vi "Run Tests in Active Project.vi"(10 "Virtual Folder (empty: \"My Computer\")":string) -> ()   [LabVIEW 2020]
uses:
  subVIs/Run Tests (Project).vi
  Caraya.lvlib
panel:
  out "error out":errorcluster
  # "CARAYA Run Active Project's Unit Tests\n\nThis tool will run all Caraya Unit Tests found in the active project."
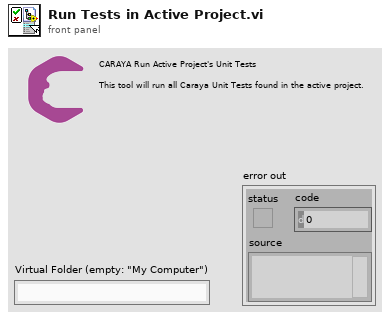
[diagram p1: front panel]
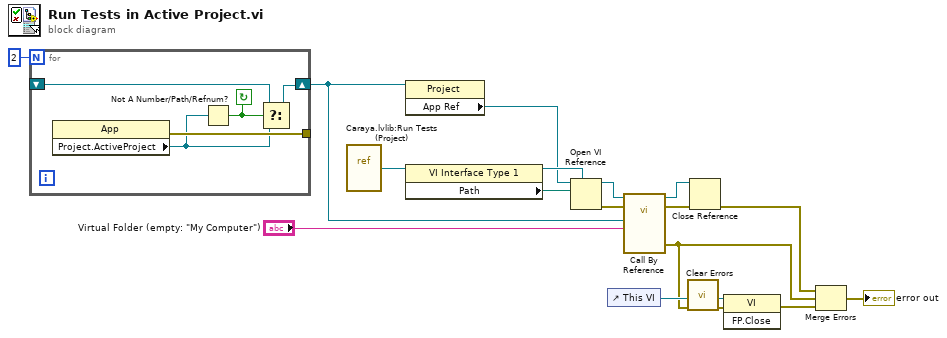
[diagram p0: block diagram]
diagram:
  n1 = for {
    N: 2 -> [_]
    tunnel: [w22] -> _
    shift-right: [w19] -> w1
    shift-left: _ -> [w20]
    stop <- w18 continue-if-true
    n2 = property on="Property Node" class="App"() -> (error out=w22:errorcluster, "Project.ActiveProject"=w21:refnum<vi>)  [unwired: 2 in, 1 out]
    n3 = Not A Number/Path/Refnum?(number/path/refnum=w21) -> (NaN/Path/Refnum?=w18:bool)
    n4 = Select(t=w20, s=w18, f=w21) -> (s? t:f=w19:refnum<vi>)
  }
  n5 = vi-ref "Caraya.lvlib:Run Tests (Project).vi"() -> (w10:refnum<vi>)
  n6 = property class="Project"(reference=w1) -> ("App Ref"=w2:refnum<vi>)  [unwired: 1 in, 2 out]
  n7 = property class="VI Interface Type 1"(reference=w10) -> (reference out=w9:refnum<vi>, "Path"=w8:path)  [unwired: 1 in, 1 out]
  n8 = Open VI Reference(type specifier VI Refnum (for type only)=w9, application reference (local)=w2, vi path=w8) -> (vi reference=w6:refnum<vi>, error out=w7:errorcluster)  [unwired: 3 in]
  n9 = control-ref of="This VI"() -> (w15:refnum<vi>)
  n10 = call-by-ref "?"(reference=w6, error in=w7, "Virtual Folder (empty: \"My Computer\")"="Virtual Folder (empty: \"My Computer\")", "Project"=w1) -> (reference out=w4:refnum<vi>, error out=w5:errorcluster, 0:"error out"=w12:errorcluster)  [unwired: 9 in]
  n11 = call <vilib>:"Clear Errors.vi"("error in (no error)"=w12) -> ("error out"=w13:errorcluster)  [unwired: 5 in, 1 out]
  n12 = Close Reference(reference=w4, error in (no error)=w5) -> (error out=w3:errorcluster)
  n13 = invoke class="VI" method="FP.Close"(reference=w15, error in=w13) -> (error out=w14:errorcluster)  [unwired: 1 in, 2 out]
  n14 = Merge Errors(w3, w12, w14) -> (→"error out":errorcluster)
